vi "DetermineCommandLineArgs.vi"(10 "CLI Arguments":string[](array[string]), 11 "App.Args in":string[](array[string])) -> (3 "App.Args out":string[](array[string]))   [LabVIEW 2019, in "SolutionBuilder.lvlib"]
uses:
  SolutionBuilder/SolutionBuilder.lvlib
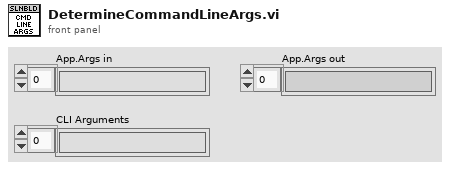
[diagram p1: front panel]
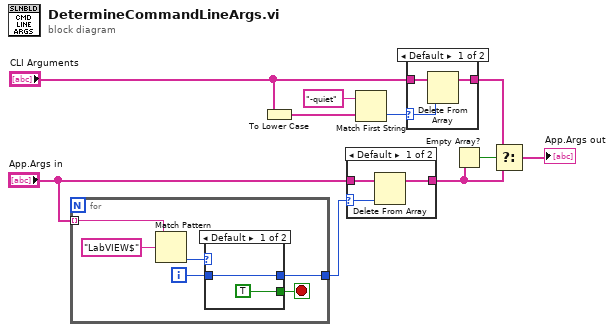
[diagram p0: block diagram]
diagram:
  n1 = for {
    tunnel: [w12] -> w10
    tunnel: "App.Args in" -> [w15] mode=indexing
    i -> [w13]
    stop <- w11 stop-if-true
    n2 = Match Pattern(string=w15, regular expression="LabVIEW$" ("string")) -> (offset past match=w14:i32)  [unwired: 1 in, 3 out]
    n3 = case shown="Default" w14 {
      selector: w14 -> [_ w19]
      tunnel: w13 -> [w18 _]
      tunnel: [w18 w19] -> w12
      tunnel: [TRUE _] -> w11
      frame Default {
      }
      frame -1 {
      }
    }
  }
  n4 = To Lower Case(string="CLI Arguments") -> (all lower case string=w5:string[])
  n5 = case shown="Default" w10 {
    selector: w10 -> [w21 _]
    tunnel: "App.Args in" -> [w22 w23]
    tunnel: [w20 w23] -> w8
    frame Default {
      n6 = Delete From Array(array=w22, index=w21) -> (array with subset deleted=w20:string[])  [unwired: 1 in, 1 out]
    }
    frame -1 {
    }
  }
  n7 = Match First String(2:w5, 3:"-quiet" ("string")) -> (0:w4:i32)  [unwired: 1 out]
  n8 = case shown="Default" w4 {
    selector: w4 -> [w25 _]
    tunnel: "CLI Arguments" -> [w26 w27]
    tunnel: [w24 w27] -> w2
    frame Default {
      n9 = Delete From Array(array=w26, index=w25) -> (array with subset deleted=w24:string[])  [unwired: 1 in, 1 out]
    }
    frame -1 {
    }
  }
  n10 = Empty Array?(array=w8) -> (empty?=w9:bool)
  n11 = Select(t=w2, s=w9, f=w8) -> (s? t:f=→"App.Args out":string[])
